vi "WLAN_SuperposedFrameBuild_V4.vi"(4 "Modulation parameter LP":T1, 6 "OFDMON":bool, 7 "Alpha":dbl min=0.0 max=1.0 step=0.05 format="%#_13g", 8 "error in (no error)":errorcluster, 9 "data in 2":i8[](array[numeric]) caption="input bit stream", 10 "Modulation parameter HP":T1, 11 "data in":i8[](array[numeric]) caption="input bit stream") -> (0 "error out":errorcluster, 3 "output array":cdb[](array[numeric]))   [LabVIEW 2022 SP3]
panel:
  out "scrambled bits":i8[](array[numeric])
  out "symbols":cdb[](array[numeric])
  out "x+y":cdb[](array[numeric])
  out "output bit stream 4":i8[](array[numeric])
  out "output bit stream 3":i8[](array[numeric])
  out "subarray 2":i8[](array[numeric])
  out "subarray":i8[](array[numeric])
  out "size(s) 2":i32
  out "size(s) 6":i32
  out "size(s) 5":i32
  out "size(s) 4":i32
  out "size(s) 3":i32
  out "size(s)":i32
  in  "data in 3":i8[](array[numeric]) caption="input bit stream"
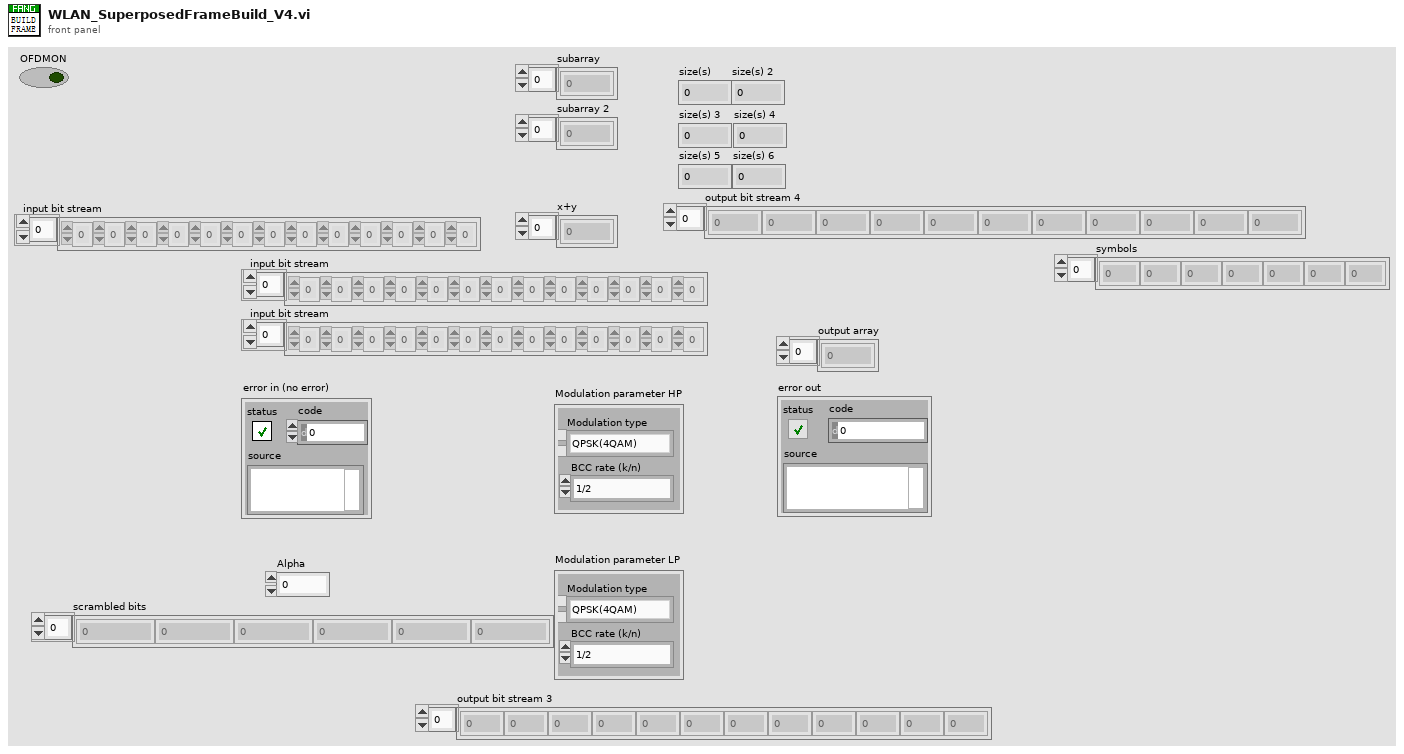
[diagram p1: front panel]
types:
  T1 = cluster{"Modulation type":enum16{"QPSK(4QAM)", "64QAM", "16QAM", "BPSK"}, "BCC rate (k/n)":enum16{"1/2", "2/3", "3/4"}}
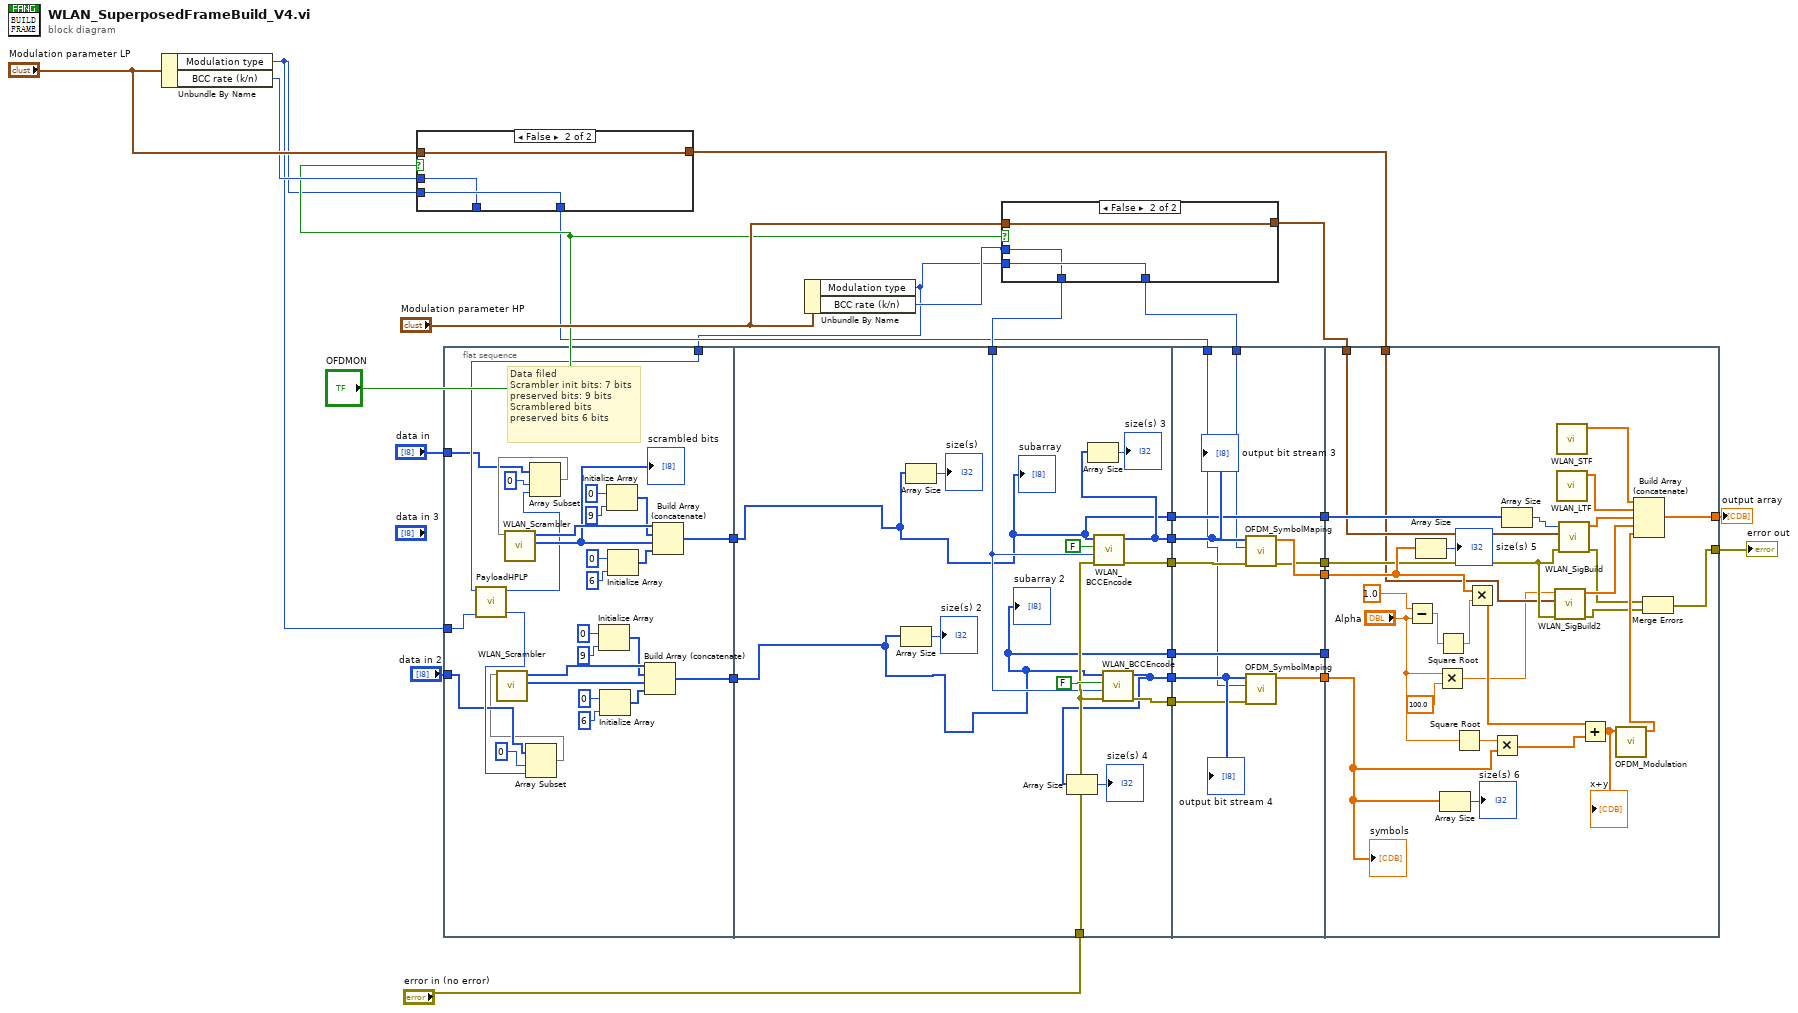
[diagram p0: block diagram]
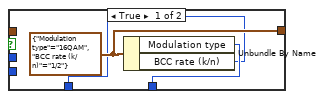
[diagram p2: hidden frame]
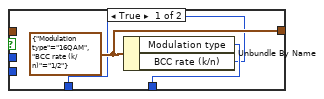
[diagram p3: hidden frame]
diagram:
  n1 = Unbundle By Name("Modulation parameter LP") -> ("Modulation type"=w2:enum16{"QPSK(4QAM)", "64QAM", "16QAM", "BPSK"}, "BCC rate (k/n)"=w6:enum16{"1/2", "2/3", "3/4"})
  n2 = case shown="False" "OFDMON" {
    tunnel: w2 -> [_ w36]
    tunnel: [w33 w36] -> w4
    tunnel: [w32 w35] -> w3
    tunnel: "Modulation parameter LP" -> [_ w35]
    tunnel: [w31 w34] -> _
    tunnel: w6 -> [_ w34]
    frame True {
      w32 = T1 {"Modulation type"=enum."16QAM", "BCC rate (k/n)"=enum."1/2"} ("Modulation parameter")
      n3 = Unbundle By Name(w32) -> ("Modulation type"=w33:enum16{"QPSK(4QAM)", "64QAM", "16QAM", "BPSK"}, "BCC rate (k/n)"=w31:enum16{"1/2", "2/3", "3/4"})
    }
    frame False {
    }
  }
  n4 = flat-sequence {
    tunnel: "data in" -> [w39]
    tunnel: [w56] -> w29
    tunnel: "data in 2" -> [w38]
    tunnel: [w47] -> w18
    tunnel: w2 -> [w46]
    tunnel: w1 -> [w45]
    tunnel: w29 -> [w66]
    tunnel: "error in (no error)" -> [w75]
    tunnel: [w77] -> w27
    tunnel: [w69] -> w26
    tunnel: w9 -> [w74]
    tunnel: [w66] -> w21
    tunnel: w18 -> [w65]
    tunnel: [w65] -> w17
    tunnel: [w68] -> w16
    tunnel: [w73] -> w14
    tunnel: w27 -> [w89]
    tunnel: w26 -> [w88]
    tunnel: w12 -> [w80]
    tunnel: [w87] -> w25
    tunnel: [w86] -> w24
    tunnel: w21 -> [w85]
    tunnel: [w85] -> w20
    tunnel: w17 -> [w83]
    tunnel: w16 -> [w84]
    tunnel: [w83] -> w15
    tunnel: w14 -> [w82]
    tunnel: [w81] -> w13
    tunnel: w4 -> [w79]
    tunnel: w11 -> [w94]
    tunnel: w25 -> [w107]
    tunnel: w24 -> [w101]
    tunnel: [w97] -> w23
    tunnel: [w114] -> w22
    tunnel: w20 -> [w96]
    tunnel: w15 -> [_]
    tunnel: w13 -> [w105]
    tunnel: w3 -> [w93]
    frame #0 {
      # "Data filed\nScrambler init bits: 7 bits\npreserved bits: 9 bits\nScramblered bits\npreserved bits 6 bits"
      n5 = call "PayloadHPLP.vi"("Modulation type LP"=w46, "Modulation type HP"=w45) -> ("Payload_LP"=w44:i32, "Payload_HP"=w41:i32)  [unwired: 8 in]
      n6 = Array Subset(array=w38, index=0, length=w44) -> (w37:i8[])
      n7 = call "WLAN_Scrambler.vi"("input bit stream"=w37) -> ("scrambled bits"=w51:i8[], "scrambler initial bit"=w55:i8[])  [unwired: 9 in]
      n8 = Array Subset(array=w39, index=0, length=w41) -> (w40:i8[])
      n9 = call "WLAN_Scrambler.vi"("input bit stream"=w40) -> ("scrambled bits"=w60:i8[], "scrambler initial bit"=w64:i8[])  [unwired: 9 in]
      "scrambled bits" <- w60
      n10 = Initialize Array(i8 0 ("element"), 9 ("dimension size")) -> (w54:i8[])
      n11 = Initialize Array(i8 0 ("element"), 6 ("dimension size")) -> (w48:i8[])
      n12 = Initialize Array(i8 0 ("element"), 9 ("dimension size")) -> (w63:i8[])
      n13 = Initialize Array(i8 0 ("element"), 6 ("dimension size")) -> (w57:i8[])
      n14 = Build Array (concatenate)(w55, w54, w51, w48) -> (w47:i8[])
      n15 = Build Array (concatenate)(w64, w63, w60, w57) -> (w56:i8[])
    }
    frame #1 {
      n16 = Array Size(array=w65) -> (size(s)=→"size(s) 2":i32)
      n17 = Array Size(array=w66) -> (size(s)=→"size(s)":i32)
      n18 = call "WLAN_BCCEncode.vi"("error in (no error)"=w75, "BCC rate (k/n)"=w74, "need add zeros?"=FALSE, "input bit stream"=w66) -> ("error out"=w77:errorcluster, "output bit stream 3"=w69:i8[])  [unwired: 6 in]
      n19 = Array Size(array=w69) -> (size(s)=→"size(s) 3":i32)
      n20 = call "WLAN_BCCEncode.vi"("error in (no error)"=w75, "BCC rate (k/n)"=w74, "need add zeros?"=FALSE, "input bit stream"=w65) -> ("error out"=w73:errorcluster, "output bit stream 3"=w68:i8[])  [unwired: 6 in]
      n21 = Array Size(array=w68) -> (size(s)=→"size(s) 4":i32)
      "subarray" <- w66
      "subarray 2" <- w65
    }
    frame #2 {
      n22 = call "OFDM_SymbolMaping.vi"("error in (no error)"=w89, "Modulation type"=w80, "input bit stream"=w88) -> ("error out"=w86:errorcluster, "symbols"=w87:cdb[])  [unwired: 7 in]
      n23 = call "OFDM_SymbolMaping.vi"("error in (no error)"=w82, "Modulation type"=w79, "input bit stream"=w84) -> ("symbols"=w81:cdb[])  [unwired: 7 in, 1 out]
      "output bit stream 3" <- w88
      "output bit stream 4" <- w84
    }
    frame #3 {
      n24 = Subtract(x=1.0, y="Alpha") -> (x-y=w110:dbl)
      n25 = Array Size(array=w107) -> (size(s)=→"size(s) 5":i32)
      n26 = Multiply(x="Alpha", y=100.0) -> (x*y=w91:dbl)
      n27 = Square Root(x=w110) -> (sqrt(x)=w111:dbl)
      n28 = Array Size(array=w105) -> (size(s)=→"size(s) 6":i32)
      n29 = Square Root(x="Alpha") -> (sqrt(x)=w112:dbl)
      n30 = Multiply(x=w107, y=w111) -> (x*y=w103:cdb[])
      n31 = Multiply(x=w112, y=w105) -> (x*y=w113:cdb[])
      n32 = Array Size(array=w96) -> (size(s)=w95:i32)
      n33 = call "WLAN_SigBuild2.vi"("Alpha"=w91, "Modulation parameter"=w93, "error in (no error)"=w101) -> ("symbols"=w100:cdb[], "error out"=w99:errorcluster)  [unwired: 6 in]
      n34 = call "WLAN_STF.vi"() -> ("STF"=w115:cdb[])  [unwired: 11 in]
      n35 = call "WLAN_LTF.vi"() -> ("LTF"=w116:cdb[])  [unwired: 11 in]
      n36 = call "WLAN_SigBuild.vi"("Data bit length"=w95, "Modulation parameter"=w94, "error in (no error)"=w101) -> ("symbols"=w117:cdb[], "error out"=w98:errorcluster)  [unwired: 6 in]
      n37 = Add(x=w103, y=w113) -> (x+y=w108:cdb[])
      "x+y" <- w108
      n38 = call "OFDM_Modulation.vi"("Input sequence"=w108) -> ("Output sequence"=w102:cdb[])  [unwired: 10 in]
      n39 = Build Array (concatenate)(w115, w116, w117, w100, w102) -> (w114:cdb[])
      n40 = Merge Errors(w98, w99) -> (w97:errorcluster)
      "symbols" <- w105
    }
  }
  n41 = Unbundle By Name("Modulation parameter HP") -> ("Modulation type"=w1:enum16{"QPSK(4QAM)", "64QAM", "16QAM", "BPSK"}, "BCC rate (k/n)"=w8:enum16{"1/2", "2/3", "3/4"})
  n42 = case shown="False" "OFDMON" {
    tunnel: w1 -> [_ w123]
    tunnel: [w120 w123] -> w12
    tunnel: [w119 w122] -> w11
    tunnel: "Modulation parameter HP" -> [_ w122]
    tunnel: [w118 w121] -> w9
    tunnel: w8 -> [_ w121]
    frame True {
      w119 = T1 {"Modulation type"=enum."16QAM", "BCC rate (k/n)"=enum."1/2"} ("Modulation parameter")
      n43 = Unbundle By Name(w119) -> ("Modulation type"=w120:enum16{"QPSK(4QAM)", "64QAM", "16QAM", "BPSK"}, "BCC rate (k/n)"=w118:enum16{"1/2", "2/3", "3/4"})
    }
    frame False {
    }
  }
  "output array" <- w22
  "error out" <- w23
